vi "Test_Game.vi"() -> ()   [LabVIEW 2026]
doc: "Game_Place_Stone / Game_Undo 테스트."
panel:
  out "error out":errorcluster
  out "Cell 7,3":enum8{"Empty", "Black", "White"}(ring)
  out "Undone":i32
  out "Last Move":T1
  out "History Size":i32
  out "Reason":T2(array[ring])
  out "Win":bool[](array[boolean])
  out "Placed":bool[](array[boolean])
  in  "Undo Count":i32
  in  "Renju":bool=TRUE
  in  "Stones":i32[](array[numeric])=[1, 2]
  in  "Cols":i32[](array[numeric])=[3, 4]
  in  "Rows":i32[](array[numeric])=[7, 7]
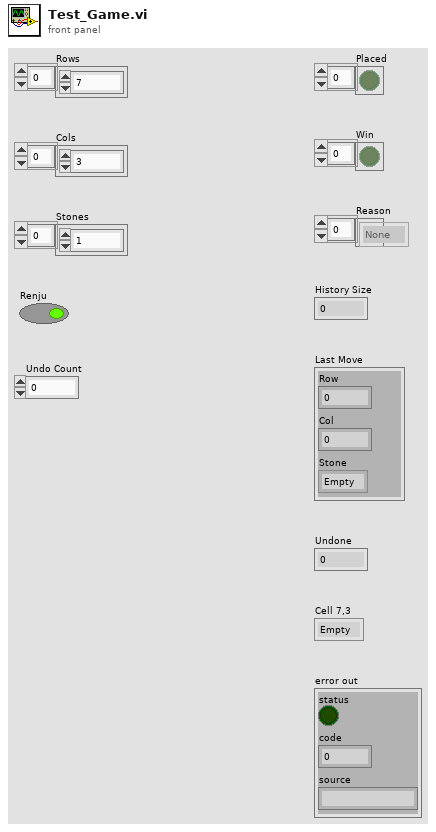
[diagram p1: front panel]
types:
  T1 = cluster{"Row":i32, "Col":i32, "Stone":enum8{"Empty", "Black", "White"}}
  T2 = enum8{"None", "Double Three", "Double Four", "Overline"}[]
  T3 = cluster{"Grid":enum8{"Empty", "Black", "White"}[][], "Move History":cluster{"Row":i32, "Col":i32, "Stone":enum8{"Empty", "Black", "White"}}[], "Last Move":cluster{"Row":i32, "Col":i32, "Stone":enum8{"Empty", "Black", "White"}}}
  T4 = enum8{"None", "Double Three", "Double Four", "Overline"}
  T5 = cluster{"Row":i32, "Col":i32, "Stone":enum8{"Empty", "Black", "White"}}[]
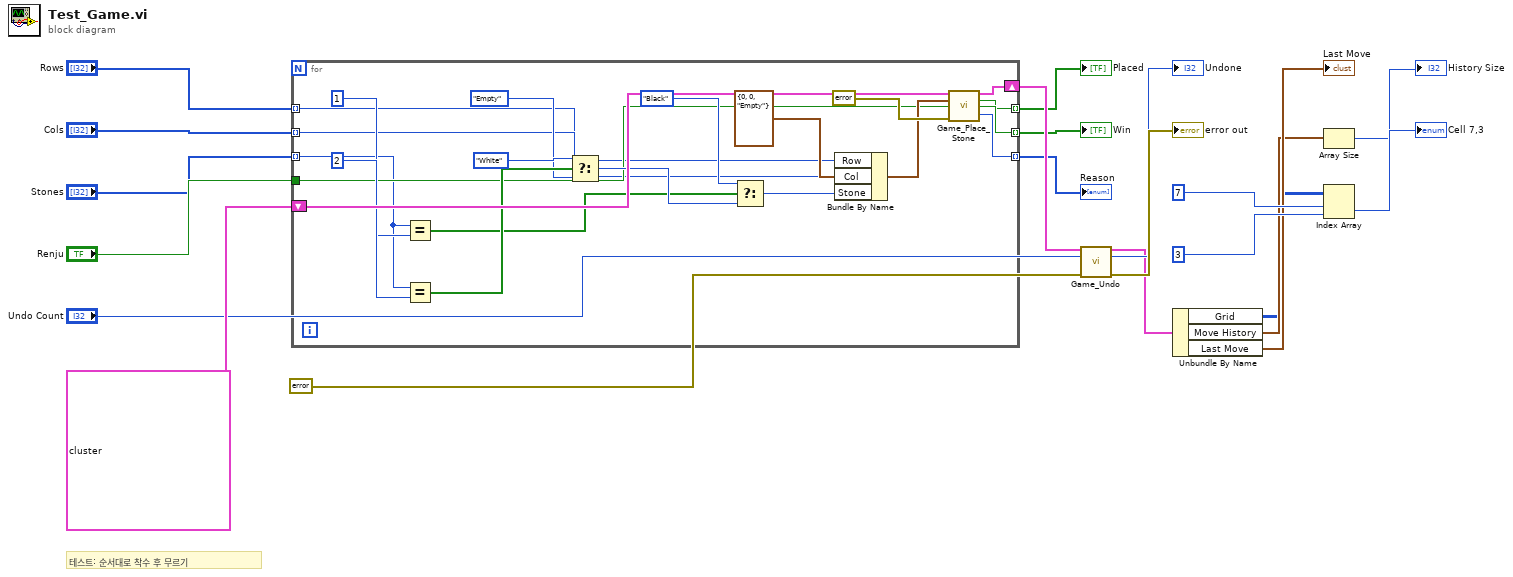
[diagram p0: block diagram]
diagram:
  # "테스트: 순서대로 착수 후 무르기"
  n1 = for {
    tunnel: "Rows" -> [w22] mode=indexing
    tunnel: "Cols" -> [w23] mode=indexing
    tunnel: "Stones" -> [w24] mode=indexing
    tunnel: "Renju" -> [w25]
    shift-right: [w38] -> w10
    shift-left: T3 {"Grid"=array15x15[225 elements], "Move History"=[], "Last Move"={"Row"=-1, "Col"=-1, "Stone"=enum."Empty"}} -> [w42]
    tunnel: [w39] -> w7 mode=indexing
    tunnel: [w40] -> w8 mode=indexing
    tunnel: [w41] -> w9 mode=indexing
    n2 = Equal?(x=w24, y=1) -> (x = y?=w31:bool[])
    n3 = Equal?(x=w24, y=2) -> (x = y?=w33:bool[])
    n4 = Select(t=enum8{"Empty", "Black", "White"}."White", s=w33, f=enum8{"Empty", "Black", "White"}."Empty") -> (s? t:f=w34:enum8{"Empty", "Black", "White"})
    n5 = Select(t=enum8{"Empty", "Black", "White"}."Black", s=w31, f=w34) -> (s? t:f=w35:enum8{"Empty", "Black", "White"})
    n6 = Bundle By Name(cluster=T1 {"Row"=0, "Col"=0, "Stone"=enum."Empty"}, "Row"=w22, "Col"=w23, "Stone"=w35) -> (w36:T1)
    n7 = call "Game_Place_Stone.vi"("Board State"=w42, "Move"=w36, "Renju"=w25, "error in"=errorcluster {"status"=FALSE, "code"=0, "source"=""}) -> ("Board State out"=w38:T3, "Placed?"=w39:bool, "Win?"=w40:bool, "Forbidden Reason"=w41:T4)  [unwired: 5 in, 3 out]
  }
  "Placed" <- w7
  "Win" <- w8
  "Reason" <- w9
  n8 = call "Game_Undo.vi"("Board State"=w10, "Count"="Undo Count", "error in"=errorcluster {"status"=FALSE, "code"=0, "source"=""}) -> ("Board State out"=w12:T3, "Undone"=→"Undone":i32, "error out"=→"error out":errorcluster)  [unwired: 10 in]
  n9 = Unbundle By Name(w12) -> ("Grid"=w15:enum8{"Empty", "Black", "White"}[][], "Move History"=w16:T5, "Last Move"=→"Last Move":T1)
  n10 = Array Size(array=w16) -> (size(s)=→"History Size":i32)
  n11 = Index Array(array=w15, index (row)=7, index (col)=3) -> (element=→"Cell 7,3":enum8{"Empty", "Black", "White"})
